vi "Test Local Queue Connection.vi"() -> ()   [LabVIEW 2013]
uses:
  <vilib>/LabVIEW Open Source Project/MQTT LocalQueue Connection/MQTT_LocalQueue/Connection/LocalQueueConnection.lvclass
  <vilib>/LabVIEW Open Source Project/Connection/Connection/Connection.lvclass
panel:
  out "value":dbl
  out "listener error":errorcluster
  out "client session error":errorcluster
  out "server session error":errorcluster
  out "Bytes":u8[](array[numeric]) format="%08b"
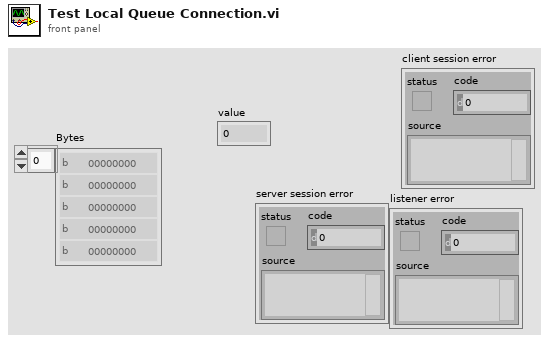
[diagram p1: front panel]
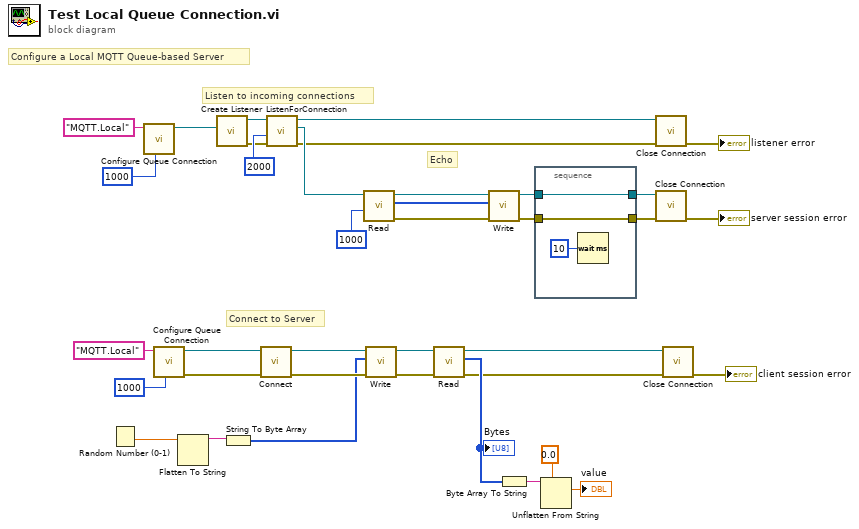
[diagram p0: block diagram]
diagram:
  # "Connect to Server"
  # "Echo"
  # "Listen to incoming connections"
  # "Configure a Local MQTT Queue-based Server"
  n1 = Random Number (0-1)() -> (number: 0 to 1=w18:dbl)
  n2 = call <vilib>:"Configure Queue Connection.vi"("timeout (500 ms)"=1000 ("timeout (100ms)"), "Queue Name"="MQTT.Local") -> ("LocalQueueConnection"=w32:refnum<class "LocalQueueConnection.lvclass">)  [unwired: 8 in, 1 out]
  n3 = call <vilib>:"Configure Queue Connection.vi"("timeout (500 ms)"=1000 ("timeout (100ms)"), "Queue Name"="MQTT.Local") -> ("error out"=w20:errorcluster, "LocalQueueConnection"=w26:refnum<class "LocalQueueConnection.lvclass">)  [unwired: 8 in]
  n4 = Flatten To String(anything=w18) -> (data string=w17:string)  [unwired: 3 in, 2 out]
  n5 = call <vilib>:"Create Listener.vi"("Connection Configuration"=w32) -> ("error out"=w33:errorcluster, "Listener"=w36:refnum<class "LocalQueueConnection.lvclass">)  [unwired: 9 in]
  n6 = String To Byte Array(string=w17) -> (unsigned byte array=w16:u8[])
  n7 = call <vilib>:"Connect.vi"("error in (no error)"=w20, "Connection in"=w26) -> ("error out"=w21:errorcluster, "Connection out"=w25:refnum<class "LocalQueueConnection.lvclass">)  [unwired: 8 in]
  n8 = call <vilib>:"ListenForConnection.vi"("error in (no error)"=w33, "timeout (2000 ms)"=2000 ("bytes to read (100)"), "Listener"=w36) -> ("error out"=w9:errorcluster, "Connection"=w30:refnum<class "Connection.lvclass">, "Listener out"=w34:refnum<class "LocalQueueConnection.lvclass">)  [unwired: 5 in, 1 out]
  n9 = call <vilib>:"Read.vi"("timeout (2000 ms)"=1000 ("bytes to read (100)"), "TCPConnection in"=w30) -> ("error out"=w23:errorcluster, "Bytes"=w28:u8[], "TCPConnection out"=w29:refnum<class "Connection.lvclass">)  [unwired: 5 in, 2 out]
  n10 = call <vilib>:"Write.vi"("error in (no error)"=w21, "Bytes"=w16, "Connection in"=w25) -> ("error out"=w22:errorcluster, "Connection"=w24:refnum<class "LocalQueueConnection.lvclass">)  [unwired: 7 in]
  n11 = call <vilib>:"Read.vi"("error in (no error)"=w22, "TCPConnection in"=w24) -> ("error out"=w7:errorcluster, "Bytes"=w15:u8[], "TCPConnection out"=w5:refnum<class "LocalQueueConnection.lvclass">)  [unwired: 5 in, 2 out]
  "Bytes" <- w15
  n12 = call <vilib>:"Write.vi"("error in (no error)"=w23, "Bytes"=w28, "Connection in"=w29) -> ("error out"=w4:errorcluster, "Connection"=w2:refnum<class "Connection.lvclass">)  [unwired: 7 in]
  n13 = Byte Array To String(unsigned byte array=w15) -> (string=w14:string)
  n14 = stacked-sequence {
    tunnel: w4 -> [w39]
    tunnel: [w39] -> w3
    tunnel: w2 -> [w38]
    tunnel: [w38] -> w1
    frame #0 {
      n15 = Wait (ms)(milliseconds to wait=u32 10) -> ()  [unwired: 1 out]
    }
  }
  n16 = Unflatten From String(type=0.0, binary string=w14) -> (value=→"value":dbl)  [unwired: 3 in, 2 out]
  n17 = call <vilib>:"Close Connection.vi"("error in (no error)"=w9, "Connection in"=w34) -> ("error out"=→"listener error":errorcluster)  [unwired: 8 in, 1 out]
  n18 = call <vilib>:"Close Connection.vi"("error in (no error)"=w3, "Connection in"=w1) -> ("error out"=→"server session error":errorcluster)  [unwired: 8 in, 1 out]
  n19 = call <vilib>:"Close Connection.vi"("error in (no error)"=w7, "Connection in"=w5) -> ("error out"=→"client session error":errorcluster)  [unwired: 8 in, 1 out]
